vi "Update Value.vi"(6 "Time":dbl, 8 "error in (no error)":errorcluster, 11 "2WayValve in":refnum<class "2WayValveV.lvclass">) -> (0 "error out":errorcluster, 1 "Update":bool, 2 "Value":variant, 3 "2WayValve out":refnum<class "2WayValveV.lvclass">)   [LabVIEW 2020, in "VolatusGUIElements.lvlib" / "2WayValveV.lvclass"]
uses:
  2WayValveV.lvclass
  2WayValveV.lvclass/2WayValveV.ctl
  Command Picture.vi
  Feedback Picture.vi
  Energized Picture.vi
  Picture.vi
  VolatusGUI/Element Inhibit/Element Inhibit.lvclass
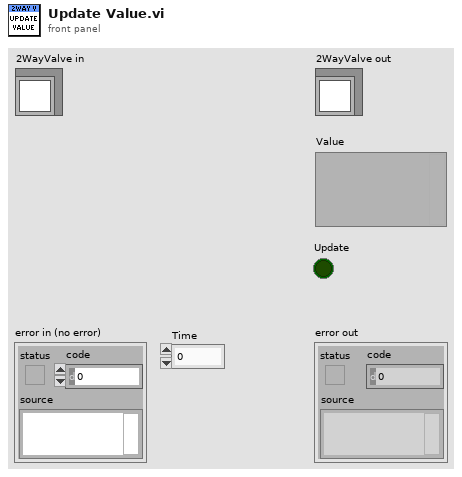
[diagram p1: front panel]
types:
  T1 = typedef "VolatusGUIElements.lvlib/2WayValveV.lvclass/Values.ctl" = cluster{"Command":T2, "CmdFB":T2, "Closed":T2, "Open":T2, "Energized":T2}
  T2 = typedef "VolatusGUIElements.lvlib/2WayValveV.lvclass/Channel State.ctl" = cluster{"Value":bool, "Stale":bool, "Config":bool, "Error":bool, "Prev":bool}
  T3 = typedef "VolatusGUIElements.lvlib/2WayValveV.lvclass/Unused Element.ctl" = cluster{"Command":bool, "Feedback":bool, "Energized":bool}
  T4 = typedef "VolatusGUIElements.lvlib/2WayValveV.lvclass/Picture.ctl" = enum16{"Blank", "OutClose", "OutOpen", "OutTranClose", "OutTranOpen", "OutConfig", "OutStale", "OutError", "InClose", "InOpen", "InTranClose", "InTranOpen", "InConfig", "InStale", "InError", "EnOff", "EnOn", "EnConfig", "EnStale", "EnError"}
  T5 = typedef "VolatusGUIElements.lvlib/2WayValveV.lvclass/Valve Pictures.ctl" = cluster{"Command":T6, "Feedback":T7, "Energized":T8}
  T6 = typedef "VolatusGUIElements.lvlib/2WayValveV.lvclass/Command Pictures.ctl" = cluster{"Error":T4, "Config":T4, "Stale":T4, "Close":T4, "Open":T4, "TranClose":T4, "TranOpen":T4}
  T7 = typedef "VolatusGUIElements.lvlib/2WayValveV.lvclass/Feedback Pictures.ctl" = cluster{"Error":T4, "Config":T4, "Stale":T4, "Closed":T4, "Open":T4, "TranClose":T4, "TranOpen":T4}
  T8 = typedef "VolatusGUIElements.lvlib/2WayValveV.lvclass/Energized Pictures.ctl" = cluster{"Error":T4, "Config":T4, "Stale":T4, "False":T4, "True":T4}
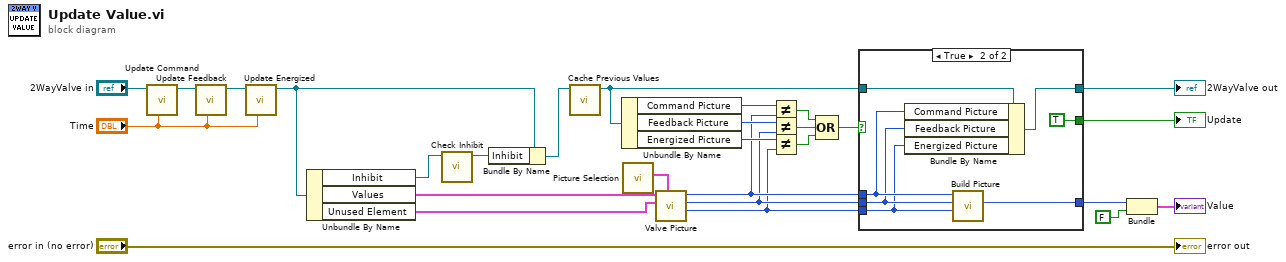
[diagram p0: block diagram]
diagram:
  n1 = call "Update Command.vi"("Time"="Time", "2WayValve in"="2WayValve in") -> ("2WayValve out"=w26:refnum<class "2WayValveV.lvclass">)  [unwired: 8 in, 1 out]
  n2 = call "Update Feedback.vi"("Time"="Time", "2WayValve in"=w26) -> ("2WayValve out"=w25:refnum<class "2WayValveV.lvclass">)  [unwired: 8 in, 1 out]
  n3 = call "Update Energized.vi"("Time"="Time", "2WayValve in"=w25) -> ("2WayValve out"=w23:refnum<class "2WayValveV.lvclass">)  [unwired: 8 in, 1 out]
  n4 = Unbundle By Name(w23) -> ("Inhibit"=w3:refnum<class "Element Inhibit.lvclass">, "Values"=w20:T1, "Unused Element"=w22:T3)
  n5 = call "Check Inhibit.vi"("Element Inhibit in"=w3) -> ("Element Inhibit out"=w1:refnum<class "Element Inhibit.lvclass">)  [unwired: 9 in, 1 out]
  n6 = Bundle By Name(cluster=w23, "Inhibit"=w1) -> (w2:refnum<class "2WayValveV.lvclass">)
  n7 = call "Cache Previous Values.vi"("2WayValve in"=w2) -> ("2WayValve out"=w11:refnum<class "2WayValveV.lvclass">)  [unwired: 9 in, 1 out]
  n8 = Unbundle By Name(w11) -> ("Command Picture"=w17:T4, "Feedback Picture"=w16:T4, "Energized Picture"=w15:T4)
  n9 = call "Picture Selection.vi"() -> ("Valve Pictures"=w21:T5)  [unwired: 11 in]
  n10 = call "Valve Picture.vi"("Valve Pictures"=w21, "Unused Element"=w22, "Values"=w20) -> ("Energized Picture"=w5:T4, "Feedback Picture"=w6:T4, "Command Picture"=w7:T4)  [unwired: 6 in]
  n11 = Not Equal?(x=w17, y=w7) -> (x != y?=w12:bool)
  n12 = Not Equal?(x=w16, y=w6) -> (x != y?=w14:bool)
  n13 = Not Equal?(x=w15, y=w5) -> (x != y?=w13:bool)
  n14 = Compound Arithmetic op=OR(w12, w14, w13) -> (w10:bool)
  n15 = case shown="True" w10 {
    tunnel: w11 -> [w29 w34]
    tunnel: [_ TRUE] -> w9
    tunnel: [_ w35] -> w8
    tunnel: w7 -> [_ w33]
    tunnel: w6 -> [_ w32]
    tunnel: w5 -> [_ w31]
    tunnel: [w29 w30] -> w4
    frame False {
    }
    frame True {
      n16 = Bundle By Name(cluster=w34, "Command Picture"=w33, "Feedback Picture"=w32, "Energized Picture"=w31) -> (w30:refnum<class "2WayValveV.lvclass">)
      n17 = call "Build Picture.vi"("Energized Picture"=w31, "Feedback Picture"=w32, "Command Picture"=w33) -> ("Valve Picture"=w35:picture)  [unwired: 8 in]
    }
  }
  "2WayValve out" <- w4
  "Update" <- w9
  n18 = Bundle("Valve Picture"=w8, FALSE) -> (→"Value":cluster{"Valve Picture":picture, bool})  [unwired: 1 in]
  "error out" <- "error in (no error)"
